vi "[ce] CalcExpress - Diagnose Script.vi"(6 "sort (F)":bool, 8 "error in":errorcluster, 9 "Items":i32(ring) items=["Variables", "Functions", "FuncVI functions", "FastFunc functions"], 10 "expression":string, 11 "CE InstanceRef":T1) -> (0 "error out":errorcluster, 1 "Array of Items":string[](array[string]), 3 "dup CE InstanceRef":T1, 4 "Original List of Items":string)   [LabVIEW 2021]
doc: "This VI returns the names of variables and functions referenced in a CalcExpress expression or sequential script. To analyze a parsed script, pass a reference to its instance context to <b>CE InstanceRef</b> control; otherwise, pass a script source to <b>expression</b> control. Refer to the VI help for more details.\n\n<b>Items</b> control defines what the VI should return.\n\n::: CalcExpress Toolkit :::\nCopyright (c) 2000-2026 Konstantin Shifershteyn. All rights reserved."
uses:
  cetypes.llb/CalcExpress Instance RefNum.ctl
  cersrc/celveng32.dll
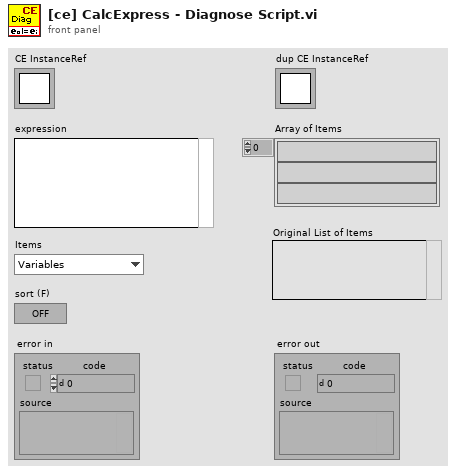
[diagram p1: front panel]
types:
  T1 = typedef "CalcExpress Instance RefNum.ctl" = refnum<k1>
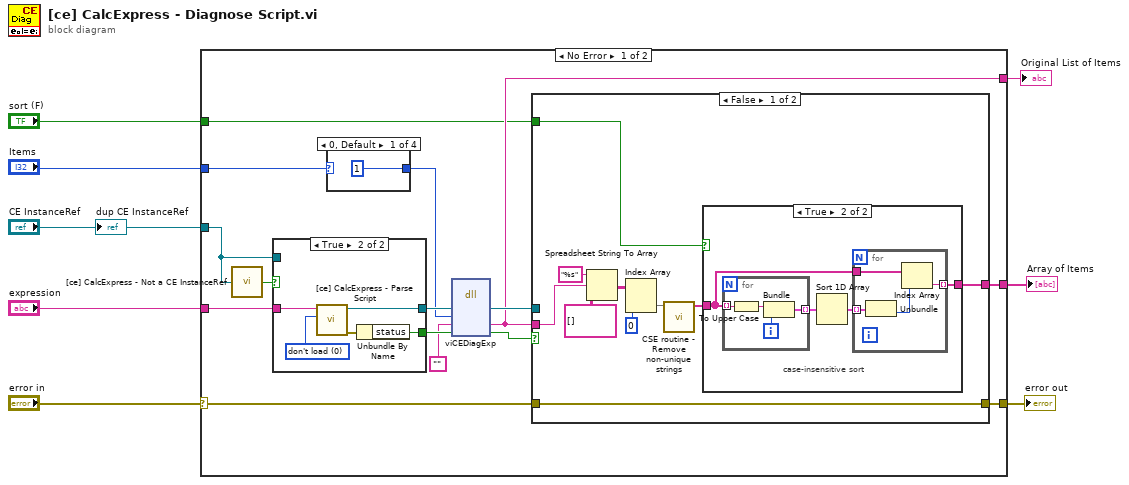
[diagram p0: block diagram]
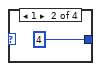
[diagram p3: hidden frame]
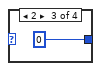
[diagram p4: hidden frame]
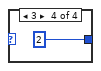
[diagram p5: hidden frame]
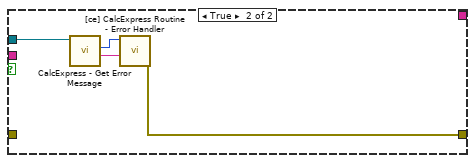
[diagram p7: hidden frame]
diagram:
  n1 = case shown="No Error" "error in" {
    selector: "error in" -> [w10 w61]
    tunnel: "expression" -> [w20 _]
    tunnel: [w18 w61] -> w7
    tunnel: [w17 _] -> w6
    tunnel: [w16 _] -> w5
    tunnel: "Items" -> [w15 _]
    tunnel: "sort (F)" -> [w13 _]
    tunnel: "CE InstanceRef" -> [w11 _]
    frame No Error {
      n2 = call "[ce] CalcExpress - Not a CE InstanceRef.vi"("CE InstanceRef"=w11) -> ("not a CE Instance"=w12:bool)  [unwired: 1 out]
      n3 = case shown="True" w12 {
        tunnel: [w24 w27] -> w23
        tunnel: [_ w25] -> w22
        tunnel: w20 -> [_ w29]
        tunnel: w11 -> [w24 _]
        frame False {
        }
        frame True {
          w28 = u32 0 items=["don't load", "load", "load & test"] ("load FuncVIs")
          n4 = call "[ce] CalcExpress - Parse Script.vi"("load FuncVIs"=w28, "expression"=w29) -> ("error out"=w26:errorcluster, "CE InstanceRef"=w27:T1)  [unwired: 4 in, 2 out]
          n5 = Unbundle By Name(w26) -> ("status"=w25:bool)
        }
      }
      n6 = case shown="0, Default" w15 {
        tunnel: [1 4 0 2] -> w14
        frame 0, Default {
        }
        frame 1 {
        }
        frame 2 {
        }
        frame 3 {
        }
      }
      n7 = dll-call lib="C:/LV Projects/CalcExpress 40 LV2021/vi.lib/addons/CalcExpress/cersrc/celveng*.dll" fn="viCEDiagExp"("iRef"=w23, "mode"=w14, "List"="", "erf"=w22) -> ("iRef"=w19:T1, "List"=w17:string, "erf"=w9:bool)  [unwired: 5 in, 2 out]
      n8 = case shown="False" w9 {
        tunnel: w10 -> [w43 _]
        tunnel: [w43 w60] -> w18
        tunnel: w19 -> [_ w58]
        tunnel: w17 -> [w36 _]
        tunnel: [w35 _] -> w16
        tunnel: w13 -> [w34 _]
        frame False {
          n9 = Spreadsheet String To Array(format string="%s", spreadsheet string=w36, array type (2D Dbl)=string[][] []) -> (array=w40:string[][])  [unwired: 1 in]
          n10 = Index Array(array=w40, index (col)=0 ("disabled index (col)")) -> (element=w42:string[])  [unwired: 1 in]
          n11 = call "CSE routine - Remove non-unique strings.vi"("Array in"=w42) -> ("Array out"=w37:string[])  [unwired: 7 in, 1 out]
          n12 = case shown="True" w34 {
            tunnel: w37 -> [w44 w46]
            tunnel: [w44 w45] -> w35
            frame False {
            }
            frame True {
              # "case-insensitive sort"
              n13 = for {
                tunnel: w46 -> [w55] mode=indexing
                tunnel: [w53] -> w48 mode=indexing
                i -> [w56]
                n14 = To Upper Case(1:w55) -> (0:w54:string)
                n15 = Bundle(w54, w56) -> (w53:cluster{string, i32})  [unwired: 1 in]
              }
              n16 = Sort 1D Array(array=w48) -> (sorted array=w47:cluster{string, i32}[])
              n17 = for {
                tunnel: w47 -> [w52] mode=indexing
                tunnel: w46 -> [w51]
                tunnel: [w49] -> w45 mode=indexing
                n18 = Unbundle(w52) -> (w50:i32)  [unwired: 1 out]
                n19 = Index Array(array=w51, index=w50) -> (element=w49:string)
              }
            }
          }
        }
        frame True {
          n20 = call "CalcExpress - Get Error Message.vi"("CE InstanceRef"=w58) -> ("error description"=w59:string, "error code"=w57:i32)  [unwired: 5 in, 2 out]
          n21 = call "[ce] CalcExpress Routine - Error Handler.vi"("error msg"=w59, "error code"=w57) -> ("error out"=w60:errorcluster)  [unwired: 7 in]
        }
      }
    }
    frame Error {
    }
  }
  "Array of Items" <- w5
  "Original List of Items" <- w6
  "error out" <- w7
  "dup CE InstanceRef" <- "CE InstanceRef"
